vi "Conformance Main.vi"(8 "error in":errorcluster) -> (0 "error out":errorcluster)   [LabVIEW 2020, in "Conformance MCP Server.lvlib"]
doc: "MCP server for the official MCP conformance suite (@modelcontextprotocol/conformance). Starts a server on http://127.0.0.1:36987/mcp/server and registers the tools, prompts and resources the suite calls by fixed names (test_simple_text, test_simple_prompt, test://static-text, ...; see Add Conformance Fixtures.vi and readme.md). Run this VI, then run tools\\test\\Invoke-Conformance.ps1. Stop ends the server; an error ends it too and is shown in a dialog."
uses:
  Conformance MCP Server.lvlib
  src/MCP Server/MCP Server.lvlib
panel:
  in  "Stop":bool
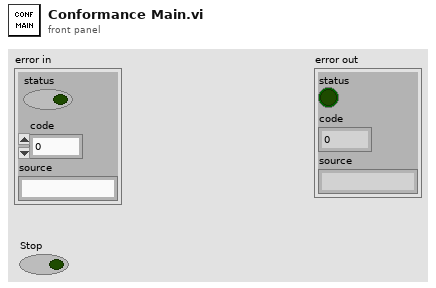
[diagram p1: front panel]
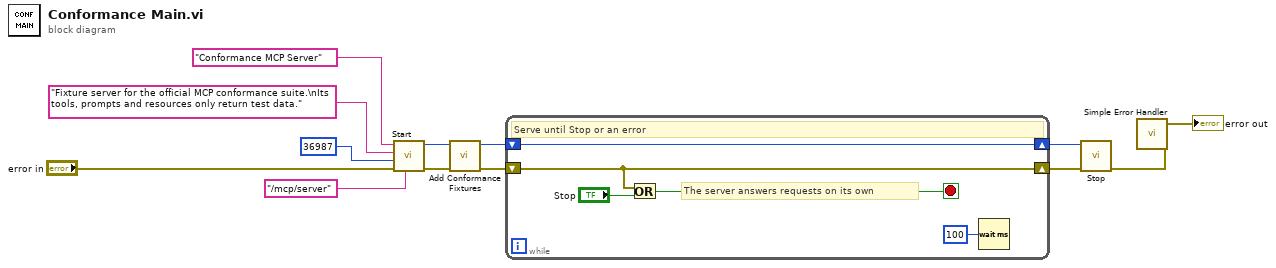
[diagram p0: block diagram]
diagram:
  n1 = call "Start.vi"("url (\"/mcp/server\")"="/mcp/server" ("url (\"/mcp/server\")"), "error in (no error)"="error in", "HTTP Port (36987)"=u16 36987, "Description"="Fixture server for the official MCP conformance suite.\nIts tools, prompts and resources only return test data.", "Name"="Conformance MCP Server") -> ("error out"=w6:errorcluster, "server id out"=w7:i32)  [unwired: 4 in, 1 out]
  n2 = call "Add Conformance Fixtures.vi"("error in"=w6, "server id"=w7) -> ("error out"=w9:errorcluster, "server id out"=w8:i32)  [unwired: 8 in]
  n3 = while {
    shift-right: [w17] -> w10
    shift-left: w9 -> [w17]
    shift-right: [w18] -> w11
    shift-left: w8 -> [w18]
    stop <- w16 stop-if-true
    # "The server answers requests on its own"
    # "Serve until Stop or an error"
    n4 = Or(x=w17, y="Stop") -> (x .or. y?=w16:bool)
    n5 = Wait (ms)(milliseconds to wait=u32 100) -> ()  [unwired: 1 out]
  }
  n6 = call "Stop.vi"("error in (no error)"=w10, "id"=w11) -> ("error out"=w12:errorcluster)  [unwired: 9 in]
  n7 = call <vilib>:"Simple Error Handler.vi"("error in (no error)"=w12) -> ("error out"=→"error out":errorcluster)  [unwired: 4 in, 4 out]
